vi "Execute.vi"(8 "error in (no error)":errorcluster, 11 "Node in":refnum<class "bt_Wait.lvclass">) -> (0 "error out":errorcluster, 1 "Status":T1, 3 "Node out":refnum<class "bt_Wait.lvclass">)   [LabVIEW 2021, in "BT.lvlib" / "bt_Wait.lvclass"]
uses:
  bt_Wait.lvclass
  abs_Node/Status.ctl
  bt_Wait.lvclass/bt_Wait.ctl
  Properties/Read Time (ms).vi
  Leaf/bt_Leaf.lvclass
  abs_Node/bt_Node.lvclass
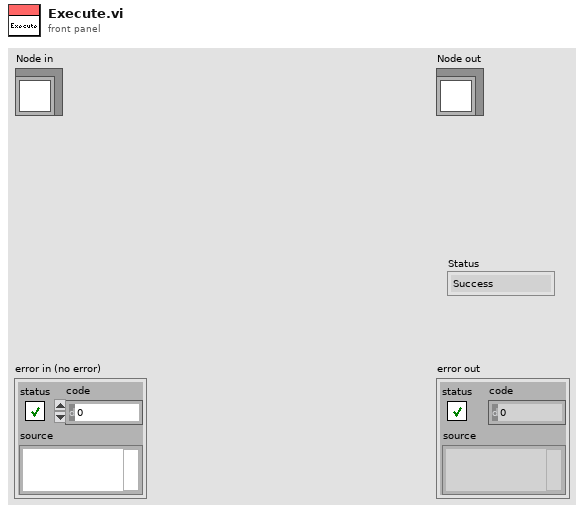
[diagram p1: front panel]
types:
  T1 = typedef "BT.lvlib/bt_Node.lvclass/Status.ctl" = enum16{"Success", "Failure", "Running"}
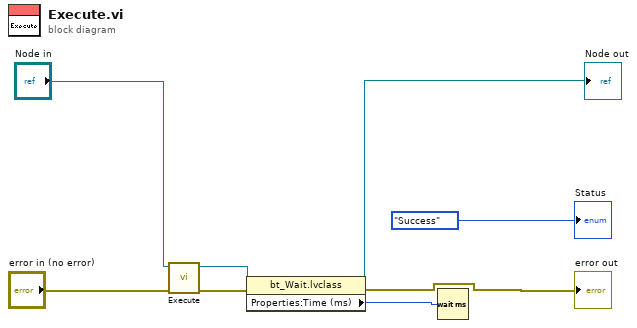
[diagram p0: block diagram]
diagram:
  n1 = call-parent "Execute.vi"("error in (no error)"="error in (no error)", "Node in"="Node in") -> ("error out"=w3:errorcluster, "Node out"=w2:refnum<class "bt_Wait.lvclass">)  [unwired: 7 in, 1 out]
  n2 = property class="bt_Wait.lvclass"(reference=w2, error in=w3) -> (reference out=→"Node out":refnum<class "bt_Wait.lvclass">, error out=→"error out":errorcluster, "Properties:Time (ms)"=w1:u32)
  n3 = Wait (ms)(milliseconds to wait=w1) -> ()  [unwired: 1 out]
  "Status" <- Status."Success" ("Status")
